vi "Method.vi"(4 "Bool":refnum<class "Abs_I8 Integer.lvclass">) -> (1 "Result":T1)   [LabVIEW 2021, in "NOT_I8.lvclass"]
uses:
  NOT_I8.lvclass
  Abs_Types/I8 Integer/Abs_I8 Integer.lvclass
  Abs_Type.ctl
  C:/Users/timst/Documents/Repositories/LV_Abstract/Source/Functions/Support/Function/One Terminal/I8/AbsFunc_One Term_I8.lvclass
  C:/Users/timst/Documents/Repositories/LV_Abstract/Source/Abs_Types/I8 Integer/Abs_I8 Integer.lvclass
  Support/Function/One Terminal/I8/AbsFunc_One Term_I8.lvclass/AbsFunc_One Term_I8.ctl
  Support/Function/One Terminal/I8/Properties/Write Numeric A.vi
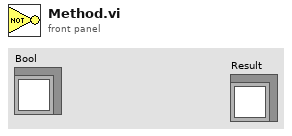
[diagram p1: front panel]
types:
  T1 = typedef "NOT_I8.lvclass/Abs_Type.ctl" = refnum<class "Abs_I8 Integer.lvclass">
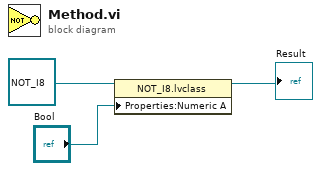
[diagram p0: block diagram]
diagram:
  n1 = property class="NOT_I8.lvclass"(reference=refnum<class "NOT_I8.lvclass"> refnum ("Functions.lvlib:Logic.lvlib:NOT.lvclass"), "Properties:Numeric A"="Bool") -> (reference out=→"Result":refnum<class "NOT_I8.lvclass">)  [unwired: 1 in, 1 out]
